vi "VI.Launch.vi"(8 "error in (no error)":errorcluster, 11 "state variables in":T4) -> (0 "error out":errorcluster, 3 "state variables out":T4)   [LabVIEW 2015, in "Multihead GUI.lvlib"]
uses:
  Multihead GUI.lvlib
  <vilib>/NI Veristand/Execution/Workspace/WorkspaceAPI.ctl
  NationalInstruments.VeriStand.ClientAPI
  <vilib>/NI Veristand/Execution/Workspace/SystemStateEventRef.ctl
  <vilib>/NI Veristand/Execution/Workspace/Target State Info.ctl
  <vilib>/NI Veristand/Execution/Workspace/Target State.ctl
  <vilib>/NI Veristand/Execution/Workspace/SystemStateRegEventRef.ctl
  <vilib>/picture/picture.llb/imagedata.ctl
  Execution GUI/Single Station Execution.lvlib
  Overview GUI/Overview GUI.lvlib
  <vilib>/NI Veristand/Execution/Workspace/NI_VS Workspace ExecutionAPI.lvlib
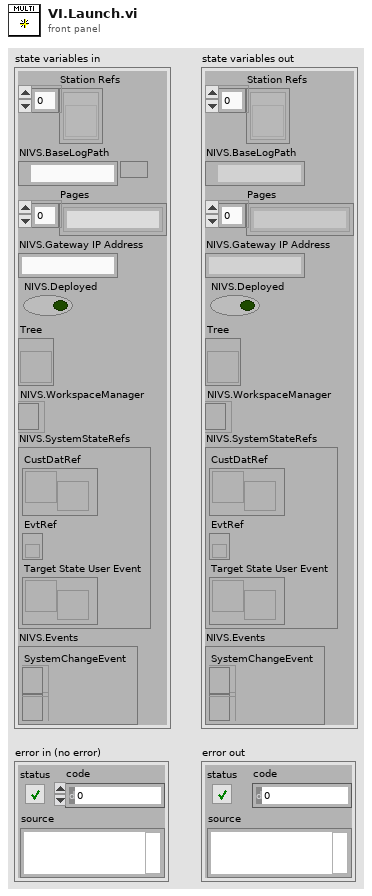
[diagram p1: front panel]
types:
  T1 = typedef "NI_VS Workspace ExecutionAPI.lvlib/WorkspaceAPI.ctl" = refnum<k24>
  T2 = typedef "NI_VS Workspace ExecutionAPI.lvlib/SystemStateEventRef.ctl" = cluster{"CustDatRef":refnum<user-event>, "EvtRef":refnum<k27>, "Target State User Event":refnum<user-event>}
  T3 = typedef "NI_VS Workspace ExecutionAPI.lvlib/SystemStateRegEventRef.ctl" = refnum<event-registration>
  T4 = cluster{"Station Refs":refnum<vi>[], "NIVS.BaseLogPath":path, "Pages":string[], "NIVS.Gateway IP Address":string, "NIVS.Deployed":bool, "Tree":refnum<vi>, "NIVS.WorkspaceManager":T1, "NIVS.SystemStateRefs":T2, "NIVS.Events":cluster{"SystemChangeEvent":T3, "WorkspaceEvent":refnum<event-registration>}}
  T5 = typedef "imagedata.ctl" = cluster{"image type":i32, "image depth":i32, "image":u8[], "mask":u8[], "colors":u32[], "Rectangle":cluster{"left":i16, "top":i16, "right":i16, "bottom":i16}}
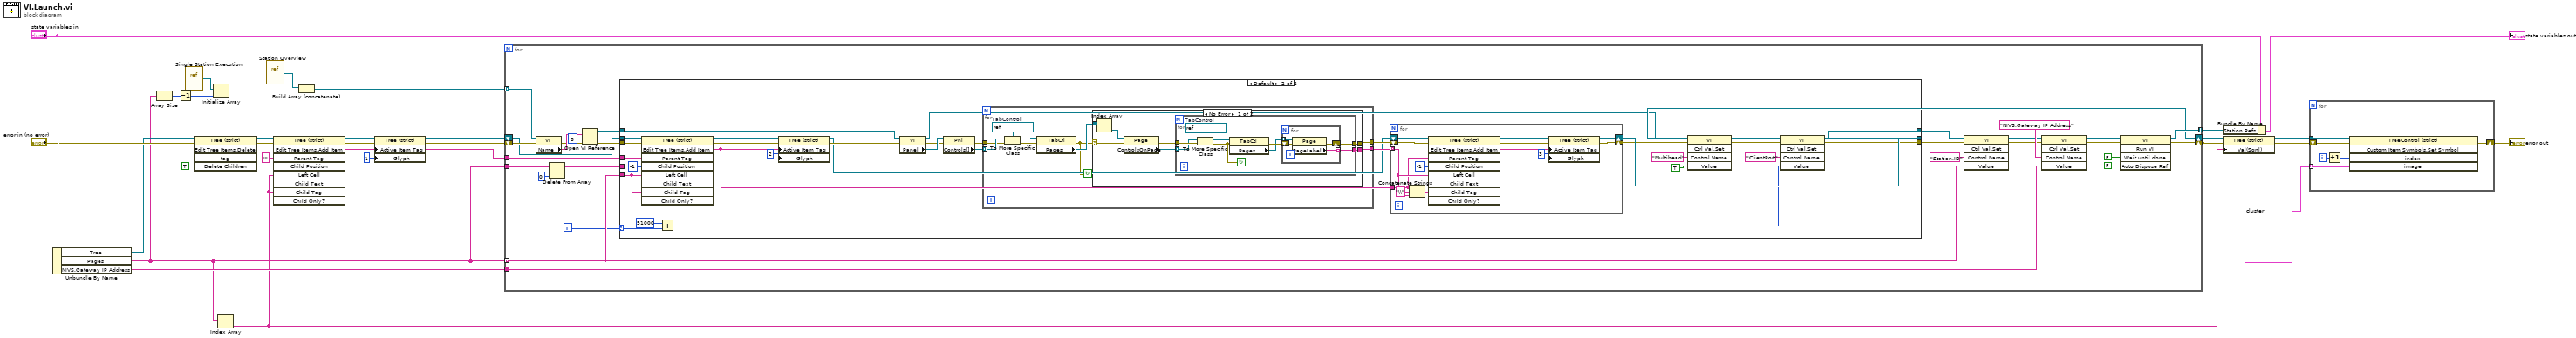
[diagram p0: block diagram]
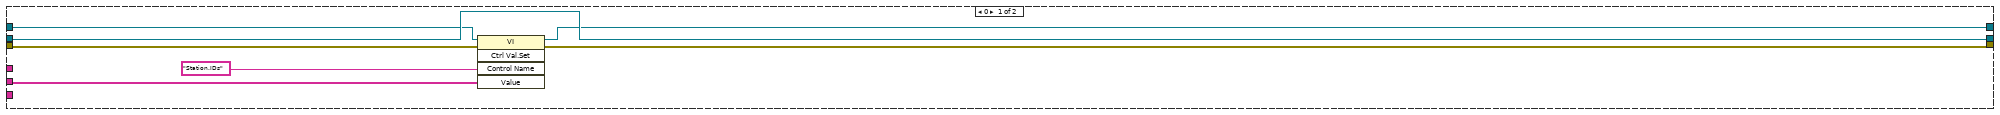
[diagram p2: hidden frame]
diagram:
  n1 = Unbundle By Name("state variables in") -> ("Tree"=w17:refnum<vi>, "Pages"=w1:string[], "NIVS.Gateway IP Address"=w30:string)
  n2 = Array Size(array=w1) -> (size(s)=w6:i32)
  n3 = Decrement(x=w6) -> (x-1=w5:i32)
  n4 = vi-ref "Single Station Execution.vi"() -> (w3:refnum<vi>)
  n5 = invoke class="Tree (strict)" method="Edit Tree Items.Delete"(reference=w17, error in="error in (no error)", "Delete Children"=TRUE ("Delete Children?")) -> (reference out=w20:refnum<vi>, error out=w21:errorcluster)  [unwired: 2 in, 3 out]
  n6 = Initialize Array(w3, w5) -> (w4:refnum<vi>[])
  n7 = Index Array(array=w1) -> (element=w2:string)  [unwired: 1 in]
  n8 = vi-ref "Station Overview.vi"() -> (w28:refnum<vi>)
  n9 = invoke class="Tree (strict)" method="Edit Tree Items.Add Item"(reference=w20, error in=w21, "Parent Tag"="", "Left Cell"=w2, "Child Tag"=w2) -> (reference out=w8:refnum<vi>, error out=w15:errorcluster, "Edit Tree Items:Add Item"=w16:string)  [unwired: 4 in, 6 out]
  n10 = Build Array (concatenate)(w28, w4) -> (w25:refnum<vi>[])
  n11 = property class="Tree (strict)"(reference=w8, error in=w15, "Active Item Tag"=w16, "Glyph"=1 ("Active Item:Symbol Index")) -> (reference out=w7:refnum<vi>, error out=w14:errorcluster)
  n12 = for {
    tunnel: w25 -> [w58] mode=indexing
    shift-right: [w55] -> w24
    shift-left: w14 -> [w39]
    tunnel: [w53] -> w26 mode=indexing
    tunnel: w1 -> [w42] mode=indexing
    tunnel: w30 -> [w46]
    tunnel: w1 -> [w45]
    tunnel: w16 -> [w43]
    shift-right: [w36] -> w18
    shift-left: w7 -> [w38]
    i -> [w37]
    n13 = property class="VI"(reference=w58, error in=w39) -> (error out=w54:errorcluster, "Name"=w57:string)  [unwired: 1 out]
    n14 = Delete From Array(array=w45, index=0) -> (array with subset deleted=w35:string[])  [unwired: 1 in, 1 out]
    n15 = Open VI Reference(vi path=w57, options=8, error in (no error)=w54) -> (vi reference=w40:refnum<vi>, error out=w41:errorcluster)  [unwired: 3 in]
    n16 = case shown="Default" w37 {
      selector: w37 -> [_ w69]
      tunnel: w43 -> [_ w96]
      tunnel: w42 -> [_ w95]
      tunnel: w41 -> [w63 w88]
      tunnel: w40 -> [w61 w87]
      tunnel: [w60 w70] -> w33
      tunnel: [w62 w72] -> w34
      tunnel: w38 -> [w65 w86]
      tunnel: [w65 w85] -> w36
      tunnel: w35 -> [w59 _]
      frame 0 {
        n17 = invoke class="VI" method="Ctrl Val.Set"(reference=w61, error in=w63, "Control Name"="Station.IDs", "Value"=w59) -> (reference out=w60:refnum<vi>, error out=w62:errorcluster)  [unwired: 1 in, 3 out]
      }
      frame Default {
        n18 = invoke class="Tree (strict)" method="Edit Tree Items.Add Item"(reference=w86, error in=w88, "Parent Tag"=w96, "Child Position"=-1, "Left Cell"=w95, "Child Tag"=w95) -> (reference out=w75:refnum<vi>, error out=w77:errorcluster, "Edit Tree Items:Add Item"=w78:string)  [unwired: 3 in, 6 out]
        n19 = Add(x=51000, y=w69) -> (x+y=w67:u16)
        n20 = property class="Tree (strict)"(reference=w75, error in=w77, "Active Item Tag"=w78, "Glyph"=2 ("Active Item:Symbol Index")) -> (reference out=w74:refnum<vi>, error out=w76:errorcluster)
        n21 = property class="VI"(reference=w87, error in=w76) -> (reference out=w81:refnum<vi>, error out=w92:errorcluster, "Panel"=w94:refnum<vi>)
        n22 = property class="Pnl"(reference=w94, error in=w92) -> (error out=w91:errorcluster, "Controls[]"=w93:refnum<vi>[])  [unwired: 1 out]
        n23 = for {
          tunnel: w93 -> [w118] mode=indexing
          tunnel: w91 -> [w116]
          tunnel: [w112] -> w90
          tunnel: [w111] -> w89
          stop <- w110 continue-if-true
          w117 = refnum<vi> refnum  # TabControl
          n24 = To More Specific Class(target class=w117, reference=w118, error in=w116) -> (specific class reference=w115:refnum<vi>, error out=w114:errorcluster)
          n25 = property class="TabCtl"(reference=w115, error in=w114) -> (error out=w110:errorcluster, "Pages"=w113:refnum<vi>[])  [unwired: 1 out]
          n26 = case shown="No Error" w110 {
            selector: w110 -> [w119 w139]
            tunnel: w113 -> [w125 _]
            tunnel: [w121 _] -> w112
            tunnel: [w120 w139] -> w111
            frame No Error {
              n27 = Index Array(array=w125) -> (element=w124:refnum<vi>)  [unwired: 1 in]
              n28 = property class="Page"(reference=w124, error in=w119) -> (error out=w123:errorcluster, "ControlsOnPage"=w122:refnum<vi>[])  [unwired: 1 out]
              n29 = for {
                tunnel: [w132] -> w121
                tunnel: [w131] -> w120
                tunnel: w123 -> [w127]
                tunnel: w122 -> [w126] mode=indexing
                stop <- w128 continue-if-true
                w134 = refnum<vi> refnum  # TabControl
                n30 = To More Specific Class(target class=w134, reference=w126, error in=w127) -> (specific class reference=w133:refnum<vi>, error out=w128:errorcluster)
                n31 = property class="TabCtl"(reference=w133, error in=w128) -> (error out=w130:errorcluster, "Pages"=w129:refnum<vi>[])  [unwired: 1 out]
                n32 = for {
                  tunnel: w129 -> [w137] mode=indexing
                  tunnel: [w136] -> w132 mode=indexing
                  shift-right: [w135] -> w131
                  shift-left: w130 -> [w138]
                  n33 = property class="Page"(reference=w137, error in=w138) -> (error out=w135:errorcluster, "PageLabel"=w136:string)  [unwired: 1 out]
                }
              }
            }
            frame Error {
            }
          }
        }
        n34 = for {
          tunnel: w90 -> [w108] mode=indexing
          shift-right: [w98] -> w82
          shift-left: w89 -> [w109]
          tunnel: w78 -> [w104]
          shift-right: [w97] -> w85
          shift-left: w74 -> [w105]
          n35 = Concatenate Strings(w104, "\\" ("string"), w108) -> (w107:string)
          n36 = invoke class="Tree (strict)" method="Edit Tree Items.Add Item"(reference=w105, error in=w109, "Parent Tag"=w104, "Child Position"=-1, "Left Cell"=w108, "Child Tag"=w107) -> (reference out=w100:refnum<vi>, error out=w99:errorcluster, "Edit Tree Items:Add Item"=w101:string)  [unwired: 3 in, 6 out]
          n37 = property class="Tree (strict)"(reference=w100, error in=w99, "Active Item Tag"=w101, "Glyph"=3 ("Active Item:Symbol Index")) -> (reference out=w97:refnum<vi>, error out=w98:errorcluster)
        }
        n38 = invoke class="VI" method="Ctrl Val.Set"(reference=w81, error in=w82, "Control Name"="Multihead", "Value"=TRUE) -> (reference out=w71:refnum<vi>, error out=w73:errorcluster)  [unwired: 1 in, 3 out]
        n39 = invoke class="VI" method="Ctrl Val.Set"(reference=w71, error in=w73, "Control Name"="ClientPort", "Value"=w67) -> (reference out=w70:refnum<vi>, error out=w72:errorcluster)  [unwired: 1 in, 3 out]
      }
    }
    n40 = invoke class="VI" method="Ctrl Val.Set"(reference=w33, error in=w34, "Control Name"="Station.ID", "Value"=w42) -> (reference out=w31:refnum<vi>, error out=w32:errorcluster)  [unwired: 1 in, 3 out]
    n41 = invoke class="VI" method="Ctrl Val.Set"(reference=w31, error in=w32, "Control Name"="NIVS.Gateway IP Address", "Value"=w46) -> (reference out=w49:refnum<vi>, error out=w48:errorcluster)  [unwired: 1 in, 3 out]
    n42 = invoke class="VI" method="Run VI"(reference=w49, error in=w48, "Wait until done"=FALSE ("Wait Until Done"), "Auto Dispose Ref"=FALSE ("Auto Dispose Reference")) -> (reference out=w53:refnum<vi>, error out=w55:errorcluster)  [unwired: 1 in, 3 out]
  }
  n43 = Bundle By Name(cluster="state variables in", "Station Refs"=w26) -> (→"state variables out":T4)
  n44 = property class="Tree (strict)"(reference=w18, error in=w24, "Val(Sgnl)"=w2) -> (reference out=w11:refnum<vi>, error out=w10:errorcluster)
  n45 = for {
    tunnel: T5[] [{"image type"=0, "image depth"=32, "image"=array[1024 elements], "mask"=[14, 0, 63, 128, 255, 224, 255, 240, 255, 240, 255, 240, 255, 248, 127, 254, 63, 255, 15, 255, 15, 255, 15, 255, 7, 255, 3, 255, 0, 254, 0, 56], "colors"=[], "Rectangle"={"left"=0, "top"=0, "right"=16, "bottom"=16}}, {"image type"=0, "image depth"=24, "image"=[255, 255, 255, 255, 255, 255, 255, 255, 255, 255, 255, 255, 255, 255, 255, 255, 255, 255, 0, 0, 255, 0, 0, 255, 255, 255, 255, 255, 0, 0, 255, 0, 0, 192, 192, 192, 255, 255, 255, 255, 255, 255, 255, 0, 0, 255, 0, 0, 255, 255, 255, 255, 255, 255, 255, 255, 255, 255, 255, 255, 255, 255, 255, 0, 0, 255, 0, 0, 255, 0, 0, 255, 255, 255, 255, 255, 0, 0, 255, 0, 0, 255, 0, 0, 192, 192, 192, 255, 0, 0, 255, 0, 0, 255, 0, 0, 255, 255, 255, 255, 255, 255, 255, 255, 255, 255, 255, 255, 0, 0, 255, 0, 0, 255, 0, 0, 255, 192, 192, 192, 255, 255, 255, 255, 255, 255, 255, 0, 0, 255, 0, 0, 255, 0, 0, 255, 0, 0, 255, 0, 0, 192, 192, 192, 0, 0, 255, 0, 0, 255, 255, 255, 255, 0, 0, 255, 0, 0, 255, 0, 0, 255, 192, 192, 192, 255, 255, 255, 255, 255, 255, 255, 255, 255, 255, 255, 255, 255, 0, 0, 255, 0, 0, 255, 0, 0, 192, 192, 192, 255, 255, 255, 0, 0, 255, 0, 0, 255, 0, 0, 255, 0, 0, 255, 0, 0, 255, 192, 192, 192, 255, 255, 255, 255, 255, 255, 255, 255, 255, 255, 255, 255, 255, 0, 0, 255, 0, 0, 255, 0, 0, 255, 0, 0, 255, 0, 0, 192, 192, 192, 255, 255, 255, 0, 0, 255, 0, 0, 255, 0, 0, 255, 192, 192, 192, 255, 255, 255, 255, 255, 255, 255, 255, 255, 255, 255, 255, 255, 0, 0, 255, 0, 0, 255, 0, 0, 192, 192, 192, 255, 0, 0, 255, 0, 0, 255, 0, 0, 255, 255, 255, 255, 255, 255, 0, 0, 255, 192, 192, 192, 255, 255, 255, 255, 255, 255, 255, 255, 255, 255, 255, 255, 255, 255, 255, 255, 0, 0, 255, 0, 0, 192, 192, 192, 255, 255, 253, 255, 255, 253, 255, 0, 0, 255, 0, 0, 255, 255, 255, 255, 255, 255, 255, 255, 255, 255, 255, 255, 0, 128, 0, 0, 128, 0, 0, 128, 0, 0, 128, 0, 0, 128, 0, 0, 128, 0, 0, 128, 0, 0, 128, 0, 0, 128, 0, 0, 0, 0, 255, 255, 255, 255, 255, 255, 255, 255, 255, 255, 255, 255, 255, 255, 255, 255, 255, 255, 0, 128, 0, 0, 128, 0, 0, 128, 0, 0, 0, 0, 255, 255, 253, 0, 128, 0, 255, 255, 253, 0, 0, 0, 0, 128, 0, 0, 0, 0, 255, 255, 255, 255, 255, 255, 255, 255, 255, 255, 255, 255, 255, 255, 255, 255, 255, 255, 0, 128, 0, 0, 128, 0, 0, 128, 0, 0, 128, 0, 0, 128, 0, 0, 128, 0, 0, 128, 0, 0, 128, 0, 0, 128, 0, 0, 0, 0, 255, 255, 255, 255, 255, 255, 255, 255, 255, 255, 255, 255, 255, 255, 255, 255, 255, 255, 0, 128, 0, 0, 0, 0, 255, 255, 253, 0, 128, 0, 0, 128, 0, 0, 0, 0, 255, 255, 253, 0, 128, 0, 0, 128, 0, 0, 0, 0, 255, 255, 255, 255, 255, 255, 255, 255, 255, 255, 255, 255, 255, 255, 255, 255, 255, 255, 0, 128, 0, 0, 128, 0, 0, 128, 0, 0, 128, 0, 0, 128, 0, 0, 128, 0, 0, 128, 0, 0, 128, 0, 0, 128, 0, 0, 0, 0, 255, 255, 255, 255, 255, 255, 255, 255, 255, 255, 255, 255, 255, 255, 255, 255, 255, 255, 0, 0, 0, 0, 0, 0, 0, 0, 0, 0, 0, 0, 0, 0, 0, 0, 0, 0, 0, 0, 0, 0, 0, 0, 0, 0, 0, 0, 0, 0, 255, 255, 255, 255, 255, 255], "mask"=[], "colors"=[], "Rectangle"={"left"=0, "top"=0, "right"=16, "bottom"=13}}, {"image type"=0, "image depth"=24, "image"=[0, 0, 0, 0, 0, 0, 0, 0, 0, 0, 0, 0, 0, 0, 0, 0, 0, 0, 0, 0, 0, 0, 0, 0, 0, 0, 0, 0, 0, 0, 0, 0, 0, 0, 0, 0, 0, 0, 0, 0, 0, 0, 255, 255, 255, 255, 255, 255, 0, 0, 0, 0, 153, 255, 0, 153, 255, 0, 153, 255, 0, 153, 255, 0, 153, 255, 0, 153, 255, 0, 153, 255, 0, 153, 255, 0, 153, 255, 0, 153, 255, 0, 153, 255, 0, 153, 255, 0, 0, 0, 255, 255, 255, 255, 255, 255, 0, 0, 0, 0, 0, 0, 0, 0, 0, 0, 0, 0, 0, 0, 0, 0, 0, 0, 0, 0, 0, 0, 0, 0, 0, 0, 0, 0, 0, 0, 0, 0, 0, 0, 0, 0, 0, 0, 0, 0, 0, 0, 255, 255, 255, 255, 255, 255, 0, 0, 0, 221, 221, 221, 221, 221, 221, 221, 221, 221, 221, 221, 221, 221, 221, 221, 221, 221, 221, 221, 221, 221, 221, 221, 221, 221, 221, 221, 221, 221, 221, 221, 221, 221, 221, 221, 221, 0, 0, 0, 255, 255, 255, 255, 255, 255, 0, 0, 0, 221, 221, 221, 221, 221, 221, 221, 221, 221, 221, 221, 221, 221, 221, 221, 221, 221, 221, 221, 221, 221, 221, 221, 221, 221, 221, 221, 221, 221, 221, 221, 221, 221, 221, 221, 221, 0, 0, 0, 255, 255, 255, 255, 255, 255, 0, 0, 0, 221, 221, 221, 221, 221, 221, 119, 119, 119, 119, 119, 119, 119, 119, 119, 0, 0, 0, 221, 221, 221, 119, 119, 119, 119, 119, 119, 119, 119, 119, 0, 0, 0, 221, 221, 221, 0, 0, 0, 255, 255, 255, 255, 255, 255, 0, 0, 0, 221, 221, 221, 221, 221, 221, 119, 119, 119, 221, 221, 221, 221, 221, 221, 0, 0, 0, 221, 221, 221, 119, 119, 119, 221, 221, 221, 221, 221, 221, 0, 0, 0, 221, 221, 221, 0, 0, 0, 255, 255, 255, 255, 255, 255, 0, 0, 0, 221, 221, 221, 221, 221, 221, 0, 0, 0, 0, 0, 0, 0, 0, 0, 0, 0, 0, 221, 221, 221, 0, 0, 0, 0, 0, 0, 0, 0, 0, 0, 0, 0, 221, 221, 221, 0, 0, 0, 255, 255, 255, 255, 255, 255, 0, 0, 0, 221, 221, 221, 221, 221, 221, 221, 221, 221, 221, 221, 221, 221, 221, 221, 221, 221, 221, 221, 221, 221, 221, 221, 221, 221, 221, 221, 221, 221, 221, 221, 221, 221, 221, 221, 221, 0, 0, 0, 255, 255, 255, 255, 255, 255, 0, 0, 0, 221, 221, 221, 221, 221, 221, 221, 221, 221, 221, 221, 221, 221, 221, 221, 221, 221, 221, 221, 221, 221, 119, 119, 119, 119, 119, 119, 119, 119, 119, 0, 0, 0, 221, 221, 221, 0, 0, 0, 255, 255, 255, 255, 255, 255, 0, 0, 0, 221, 221, 221, 221, 221, 221, 221, 221, 221, 221, 221, 221, 221, 221, 221, 221, 221, 221, 221, 221, 221, 119, 119, 119, 221, 221, 221, 221, 221, 221, 0, 0, 0, 221, 221, 221, 0, 0, 0, 255, 255, 255, 255, 255, 255, 0, 0, 0, 221, 221, 221, 221, 221, 221, 221, 221, 221, 221, 221, 221, 221, 221, 221, 221, 221, 221, 221, 221, 221, 0, 0, 0, 0, 0, 0, 0, 0, 0, 0, 0, 0, 221, 221, 221, 0, 0, 0, 255, 255, 255, 255, 255, 255, 0, 0, 0, 221, 221, 221, 221, 221, 221, 221, 221, 221, 221, 221, 221, 221, 221, 221, 221, 221, 221, 221, 221, 221, 221, 221, 221, 221, 221, 221, 221, 221, 221, 221, 221, 221, 221, 221, 221, 0, 0, 0, 255, 255, 255, 255, 255, 255, 0, 0, 0, 221, 221, 221, 221, 221, 221, 221, 221, 221, 221, 221, 221, 221, 221, 221, 221, 221, 221, 221, 221, 221, 221, 221, 221, 221, 221, 221, 221, 221, 221, 221, 221, 221, 221, 221, 221, 0, 0, 0, 255, 255, 255, 255, 255, 255, 0, 0, 0, 0, 0, 0, 0, 0, 0, 0, 0, 0, 0, 0, 0, 0, 0, 0, 0, 0, 0, 0, 0, 0, 0, 0, 0, 0, 0, 0, 0, 0, 0, 0, 0, 0, 0, 0, 0, 0, 0, 0, 255, 255, 255, 255, 255, 255, 255, 255, 255, 255, 255, 255, 255, 255, 255, 255, 255, 255, 255, 255, 255, 255, 255, 255, 255, 255, 255, 255, 255, 255, 255, 255, 255, 255, 255, 255, 255, 255, 255, 255, 255, 255, 255, 255, 255, 255, 255, 255, 255, 255, 255, 255, 255, 255], "mask"=[], "colors"=[], "Rectangle"={"left"=0, "top"=0, "right"=16, "bottom"=16}}] ("Array") -> [w145] mode=indexing
    tunnel: w11 -> [w143]
    shift-right: [w141] -> w9
    shift-left: w10 -> [w142]
    i -> [w144]
    n46 = Increment(x=w144) -> (x+1=w140:i32)
    n47 = invoke on="Invoke Node" class="TreeControl (strict)" method="Custom Item Symbols.Set Symbol"(reference=w143, error in=w142, "index"=w140, "image"=w145) -> (error out=w141:errorcluster)  [unwired: 1 in, 4 out]
  }
  "error out" <- w9
